vi "ActionVIOnDownload - Set Scan Rate.vi"(5 "System Definition Dir":path, 6 "IP address":string, 7 "Details Ref":refnum<vi>, 8 "error in":errorcluster, 10 "WebDAV session in":T1, 11 "Device Item Ref in":T2 format="%.0x") -> (0 "error out":errorcluster, 2 "WebDAV session out":T1, 3 "Device Item Ref out":T2 format="%.0x")   [LabVIEW 2024, in "SEECD System Explorer.lvlib"]
uses:
  SEECD System Explorer.lvlib
  <vilib>/NI VeriStand/Custom Device API/Custom Device Item Ref.ctl
  <vilib>/WebDAVClient/Advanced/SessionHandle.ctl
  <vilib>/NI VeriStand/Custom Device API/Custom Device API.lvlib
  <vilib>/WebDAVClient/NI_WebDAV.lvlib
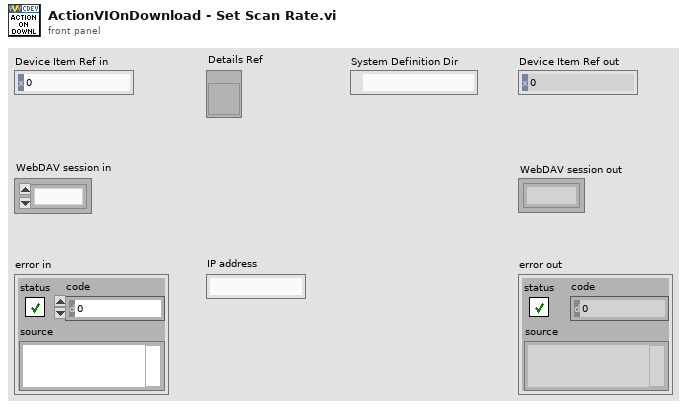
[diagram p1: front panel]
types:
  T1 = typedef "NI_WebDAV.lvlib/SessionHandle.ctl" = refnum<k1>
  T2 = typedef "Custom Device API.lvlib/Custom Device Item Ref.ctl" = u64
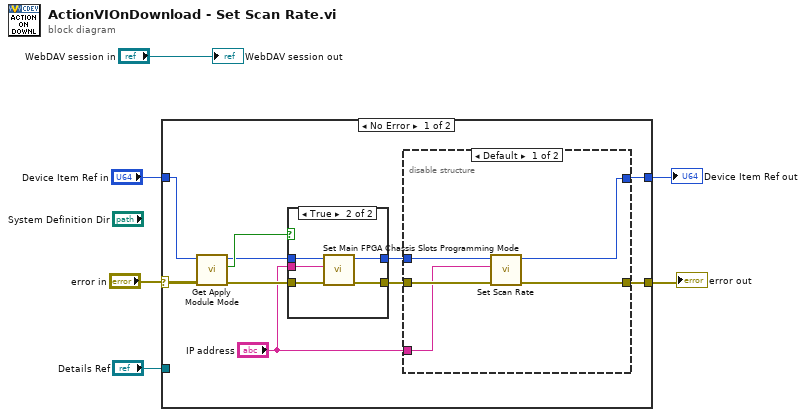
[diagram p0: block diagram]
diagram:
  n1 = case shown="No Error" "error in" {
    selector: "error in" -> [w14 w32]
    tunnel: [w16 w32] -> w5
    tunnel: "Device Item Ref in" -> [w10 w31]
    tunnel: [w7 w31] -> w1
    tunnel: "Details Ref" -> [_ _]
    frame No Error {
      n2 = call "Get Apply Module Mode.vi"("error in (no error)"=w14, "Device Item Ref in"=w10) -> ("error out"=w13:errorcluster, "Apply Module Mode"=w9:bool, "Device Item Ref out"=w8:T2)  [unwired: 7 in]
      n3 = case shown="True" w9 {
        tunnel: w8 -> [w24 w28]
        tunnel: "IP address" -> [_ w27]
        tunnel: [w25 w30] -> w15
        tunnel: [w24 w26] -> w11
        tunnel: w13 -> [w25 w29]
        frame False {
        }
        frame True {
          n4 = call "Set Main FPGA Chassis Slots Programming Mode.vi"("error in (no error)"=w29, "serverName in"=w27, "Item Ref in"=w28) -> ("error out"=w30:errorcluster, "Item Ref out"=w26:T2)  [unwired: 6 in, 1 out]
        }
      }
      n5 = disable-structure shown="Default" {
        disable-tunnel: "IP address" -> [w19 _]
        disable-tunnel: [w21 w23] -> w16
        disable-tunnel: w15 -> [w20 w23]
        disable-tunnel: w11 -> [w18 w22]
        disable-tunnel: [w17 w22] -> w7
        frame condition #0 (active) {
          n6 = call "Set Scan Rate.vi"("error in"=w20, "IP address"=w19, "Item Ref in"=w18) -> ("error out"=w21:errorcluster, "Item Ref out"=w17:T2)  [unwired: 7 in]
        }
        frame condition #1 {
        }
      }
    }
    frame Error {
    }
  }
  "error out" <- w5
  "Device Item Ref out" <- w1
  "WebDAV session out" <- "WebDAV session in"
